vi "RDV-togglePlotVisibility.vi"(8 "error in (no error)":errorcluster, 11 "RDV-Reflection_Data_viewer in":refnum<class "RDV-Reflection_Data_viewer.lvclass">) -> (0 "error out":errorcluster, 3 "RDV-Reflection_Data_viewer out":refnum<class "RDV-Reflection_Data_viewer.lvclass">)   [LabVIEW 2020, in "RDV-Reflection_Data_viewer.lvclass"]
doc: "Toggles the visibility of plots on the viewer's graphs."
uses:
  RDV-Reflection_Data_viewer.lvclass
  RDV-Reflection_Data_viewer.lvclass/RDV-Reflection_Data_viewer.ctl
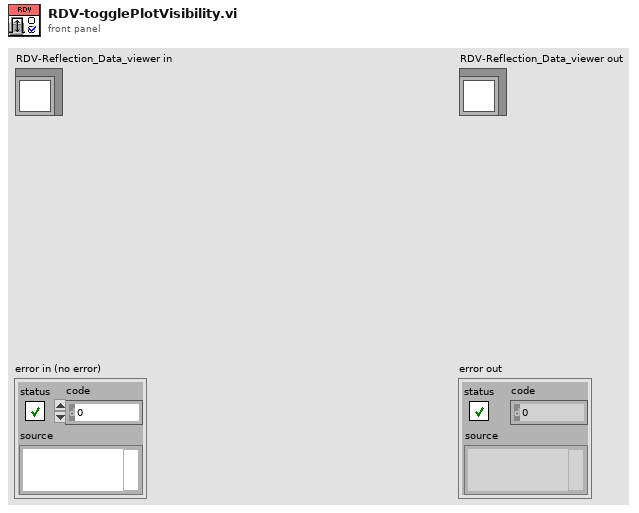
[diagram p1: front panel]
types:
  T1 = typedef "RDV-Reflection_Data_viewer.lvclass/RDV-XY_GRAPH_REFS.ctl" = cluster{"Reflection Real":refnum<vi>, "Reflection Imag":refnum<vi>, "Permittivity Real":refnum<vi>, "Permittivity Imag":refnum<vi>, "Impedance Real":refnum<vi>, "Impedance Imag":refnum<vi>}
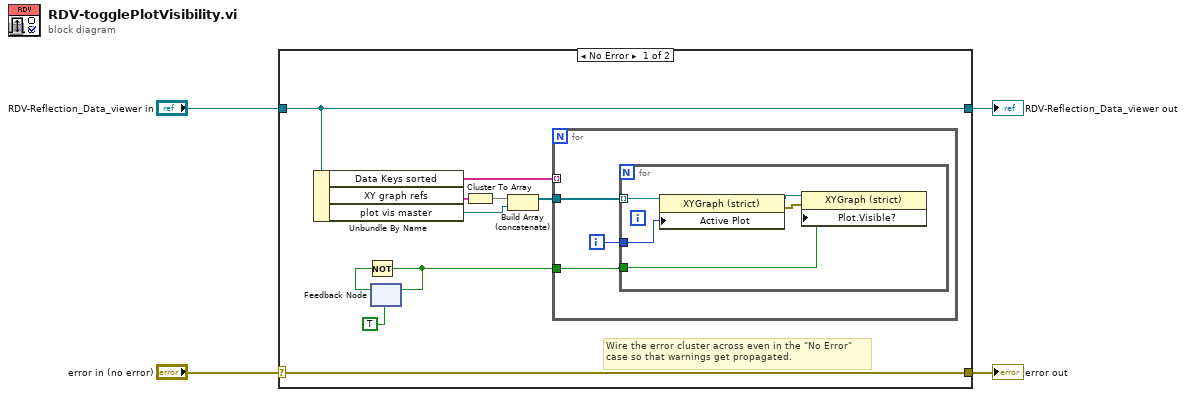
[diagram p0: block diagram]
diagram:
  n1 = case shown="No Error" "error in (no error)" {
    selector: "error in (no error)" -> [w14 w24]
    tunnel: [w14 w24] -> w3
    tunnel: [w11 w23] -> w1
    tunnel: "RDV-Reflection_Data_viewer in" -> [w11 w23]
    frame No Error {
      # "Wire the error cluster across even in the \"No Error\"\ncase so that warnings get propagated."
      n2 = Unbundle By Name(w11) -> ("Data Keys sorted"=w8:string[], "XY graph refs"=w9:T1, "plot vis master"=w5:refnum<vi>)
      n3 = feedback #1(TRUE) -> (w12:bool)
      n4 = Not(x=w12) -> (.not. x?=w10:bool)
      n5 = feedback-in #1(w10) -> ()
      n6 = Cluster To Array(cluster=w9) -> (array=w7:refnum<vi>[])
      n7 = Build Array (concatenate)(w7, w5) -> (w6:refnum<vi>[])
      n8 = for {
        tunnel: w10 -> [w17]
        tunnel: w6 -> [w16]
        tunnel: w8 -> [_] mode=indexing
        i -> [w15]
        n9 = for {
          tunnel: w17 -> [w22]
          tunnel: w16 -> [w21] mode=indexing
          tunnel: w15 -> [w18]
          n10 = property on="Property Node" class="XYGraph (strict)"(reference=w21, "Active Plot"=w18) -> (reference out=w20:refnum<vi>, error out=w19:errorcluster)  [unwired: 1 in]
          n11 = property on="Property Node" class="XYGraph (strict)"(reference=w20, error in=w19, "Plot.Visible?"=w22) -> ()  [unwired: 2 out]
        }
      }
    }
    frame Error {
    }
  }
  "error out" <- w3
  "RDV-Reflection_Data_viewer out" <- w1
